vi "Main.vi"() -> ()   [LabVIEW 2020]
panel:
  out "Application:Command Line Arguments":string[](array[string])
  in  "Start":bool
  out "current time":timestamp
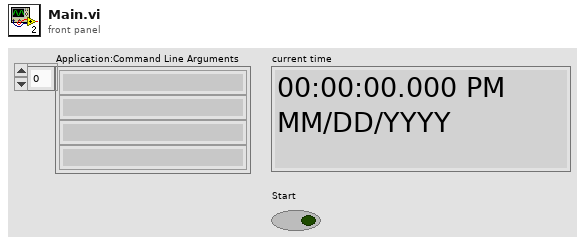
[diagram p1: front panel]
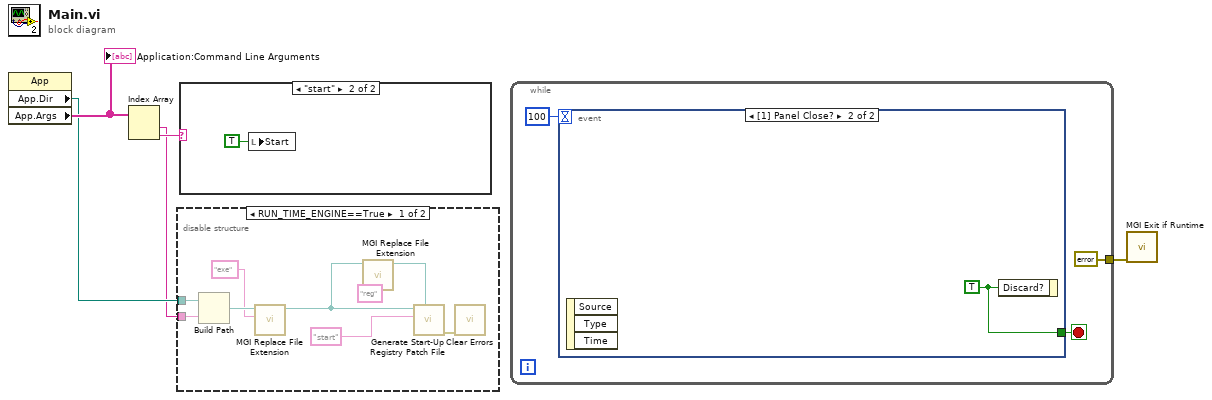
[diagram p0: block diagram]
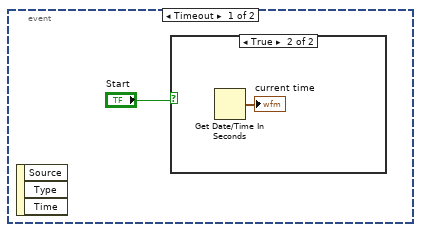
[diagram p4: hidden frame]
diagram:
  n1 = property class="App"() -> ("App.Dir"=w2:path, "App.Args"=w4:string[])  [unwired: 2 in, 2 out]
  "Application:Command Line Arguments" <- w4
  n2 = Index Array(array=w4) -> (element #1=w1:string, element #2=w3:string)  [unwired: 2 in]
  n3 = disable-structure "Conditional Disable Structure" shown="RUN_TIME_ENGINE==True" {
    disable-tunnel: w2 -> [w11 _]
    disable-tunnel: w1 -> [w10 _]
    frame condition #0 {
      n4 = Build Path(base path=w11, name or relative path=w10) -> (appended path=w9:path)
      n5 = call <userlib>:"MGI Replace File Extension.vi"("New Extension (txt)"="exe", "Path In"=w9) -> ("Path Out"=w7:path)  [unwired: 8 in, 1 out]
      n6 = call <userlib>:"MGI Replace File Extension.vi"("New Extension (txt)"="reg", "Path In"=w7) -> ("Path Out"=w12:path)  [unwired: 8 in, 1 out]
      n7 = call "Generate Start-Up Registry Patch File.vi"("RegPath"=w12, "Arguments"="start", "EXE Path"=w7) -> ("error out"=w6:errorcluster)  [unwired: 8 in]
      n8 = call <vilib>:"Clear Errors.vi"("error in (no error)"=w6) -> ()  [unwired: 5 in, 2 out]
    }
    frame condition #1 (active) {
    }
  }
  n9 = case shown="\"start\"" w3 {
    frame "False", Default {
    }
    frame "start" {
      n10 = local write "Start"(TRUE ("Start")) -> ()
    }
  }
  n11 = while {
    tunnel: [errorcluster {"status"=FALSE, "code"=0, "source"=""} ("Error In (Dependency Only)")] -> w5
    stop <- w18 stop-if-true
    n12 = event shown="[1] Panel Close?" {
      selector: _ -> [_ _]
      dyn-events: _ -> [_ _]
      timeout: 100 -> [_ _]
      tunnel: [_ w21] -> w18
      event Timeout {
        n13 = event-data() -> ()  [unwired: 1 in, 3 out]
        n14 = case shown="True" "Start" {
          frame False {
          }
          frame True {
            n15 = Get Date/Time In Seconds() -> (seconds since 1Jan1904=→"current time":timestamp)
          }
        }
      }
      event Panel Close? {
        w21 = TRUE ("Discard?")
        n16 = event-data() -> ()  [unwired: 1 in, 3 out]
        n17 = event-data("Discard?"=w21) -> ()  [unwired: 1 in, 1 out]
      }
    }
  }
  n18 = call <userlib>:"MGI Exit if Runtime.vi"("Error In (Dependency Only)"=w5) -> ()  [unwired: 11 in]
